vi "loadGraph.vi"(1 "filePath":path, 2 "graphics":refnum<class "Graphics.lvclass">, 3 "grid":refnum<class "Grid.lvclass">, 5 "error in (no error)":errorcluster) -> (14 "reference out":refnum<class "Graph.lvclass">, 15 "succeeded":bool, 16 "String":string, 17 "NodesBounds":T1 {"height" format="%.2f"; "width" format="%.2f"; "y" format="%.2f"; "x" format="%.2f"}, 19 "error out":errorcluster)   [LabVIEW 2020, in "Graph.lvclass"]
doc: "Save to File"
uses:
  <resource>/Framework/Providers/Open_GDS/UML/Graph_class/Graph.lvclass
  <resource>/Framework/Providers/Open_GDS/UML/General/Rectangle/Rectangle Rectangle2D.ctl
  <resource>/Framework/Providers/Open_GDS/UML/Grid_class/Grid.lvclass
  <resource>/Framework/Providers/Open_GDS/UML/Graphics_class/Graphics.lvclass
  <resource>/Framework/Providers/Open_GDS/UML/AbstractNode_class/AbstractNode.lvclass
  <resource>/Framework/Providers/Open_GDS/UML/AbstractEdge_class/AbstractEdge.lvclass
  <resource>/Framework/Providers/Open_GDS/UML/Graph_class/FileContent.ctl
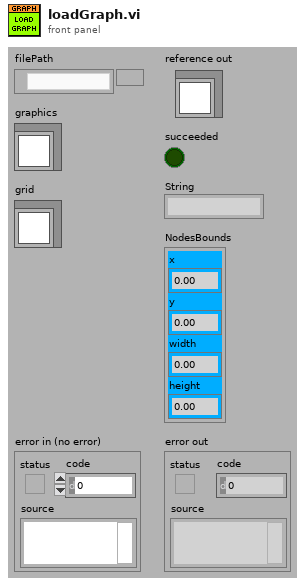
[diagram p1: front panel]
types:
  T1 = typedef "Rectangle Rectangle2D.ctl" = cluster{"x":dbl, "y":dbl, "width":dbl, "height":dbl}
  T2 = cluster{"graph":refnum<class "Graph.lvclass">, "succeeded":bool, "nodeInfo":cluster{"NodeType":string[], "ParentIndex":i32[], "ChildernIndexies":cluster{i32[]}[], "FlattenData":string[]}, "edgeInfo":cluster{"EdgeType":string[], "StartNodeIndex":i32[], "EndNodeIndex":i32[], "FlattenData":string[]}, "nodes":refnum<class "AbstractNode.lvclass">[], "edges":refnum<class "AbstractEdge.lvclass">[], "DiagramData":string, "bounds":T1, "diagramType":string}
  T3 = typedef "Graph.lvclass/FileContent.ctl" = cluster{"Version":string, "DiagramType":string, "DiagramData":string, "Nodes":cluster{"NodeType":string[], "ParentIndex":i32[], "ChildernIndexies":cluster{i32[]}[], "FlattenData":string[]}, "Edges":cluster{"EdgeType":string[], "StartNodeIndex":i32[], "EndNodeIndex":i32[], "FlattenData":string[]}}
  T4 = enum16{"read/write", "read-only", "write-only", "write-only (truncate)"}
  T5 = enum16{"None", "Class", "Sequency", "State", "UseCase"}
  T6 = cluster{"NodeType":string[], "ParentIndex":i32[], "ChildernIndexies":cluster{i32[]}[], "FlattenData":string[]}
  T7 = cluster{"EdgeType":string[], "StartNodeIndex":i32[], "EndNodeIndex":i32[], "FlattenData":string[]}
  T8 = cluster{"TYPEDEF-FileSaveVersion":enum16{"A"}, "diagramType":enum16{"None", "Class", "Sequency", "State", "UseCase"}, string, "nodeInfo":cluster{"NodeType":string[], "ParentIndex":i32[], "ChildernIndexies":cluster{i32[]}[], "FlattenData":string[]}, "edgeInfo":cluster{"EdgeType":string[], "StartNodeIndex":i32[], "EndNodeIndex":i32[], "FlattenData":string[]}}
  T9 = cluster{"diagramType":enum16{"None", "Class", "Sequency", "State", "UseCase"}, "nodeInfo":cluster{"NodeType":string[], "ParentIndex":i32[], "ChildernIndexies":cluster{i32[]}[], "FlattenData":string[]}, "edgeInfo":cluster{"EdgeType":string[], "StartNodeIndex":i32[], "EndNodeIndex":i32[], "FlattenData":string[]}}
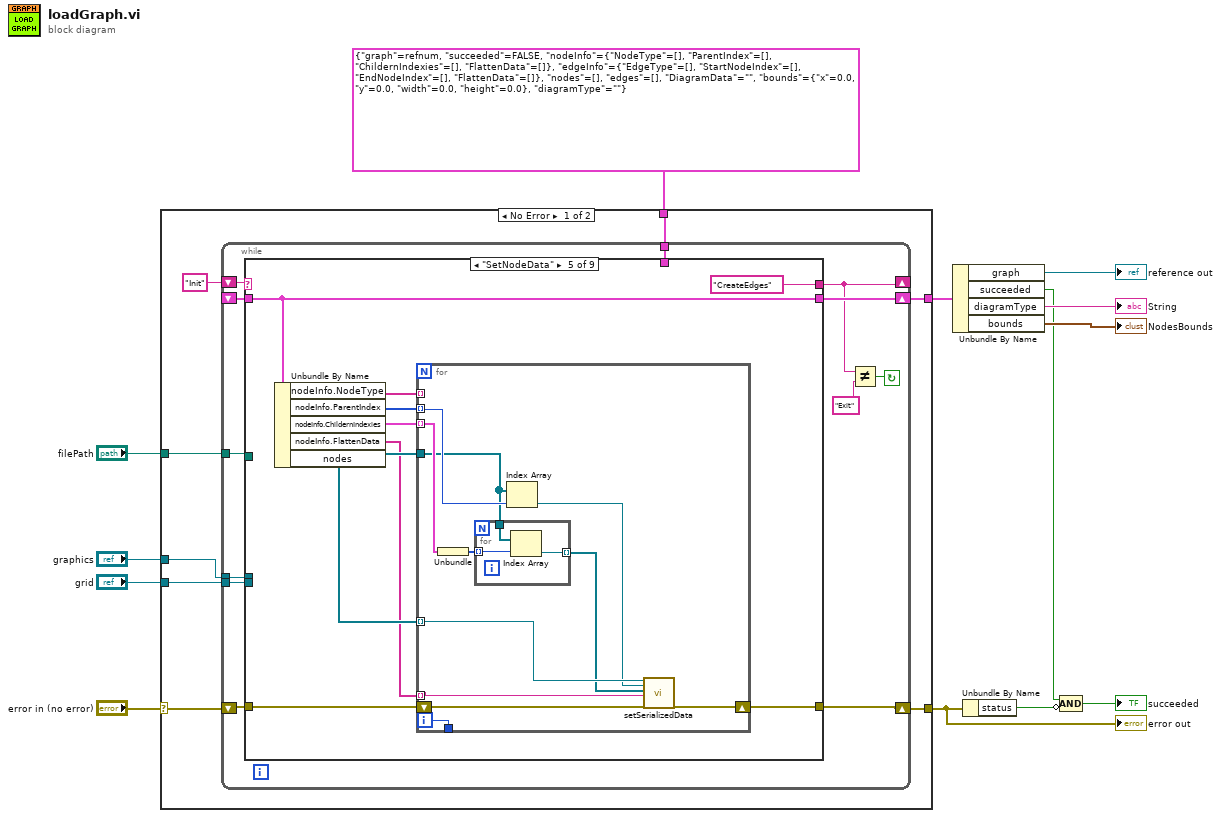
[diagram p0: block diagram]
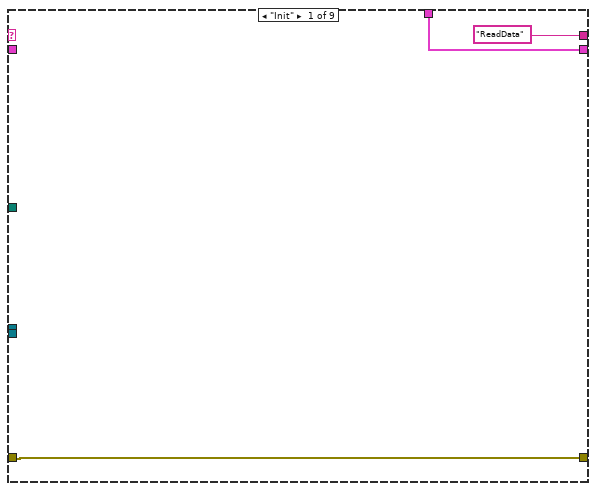
[diagram p2: hidden frame]
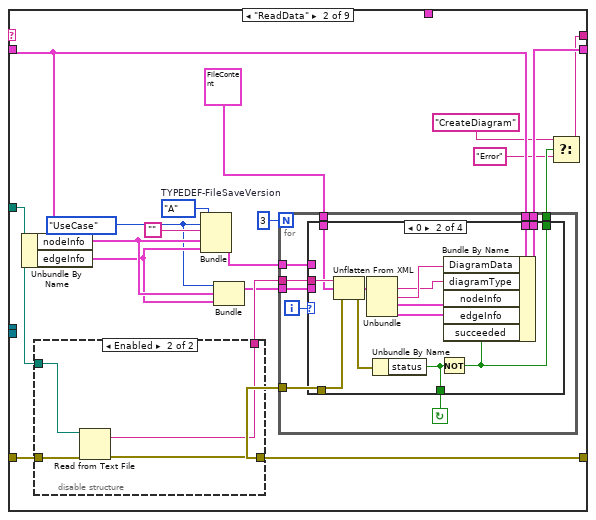
[diagram p3: hidden frame]
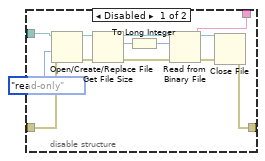
[diagram p4: hidden frame]
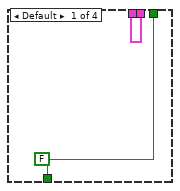
[diagram p5: hidden frame]
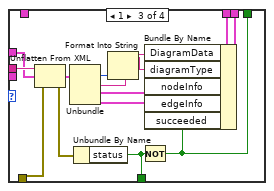
[diagram p6: hidden frame]
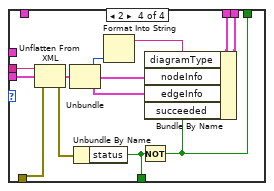
[diagram p7: hidden frame]
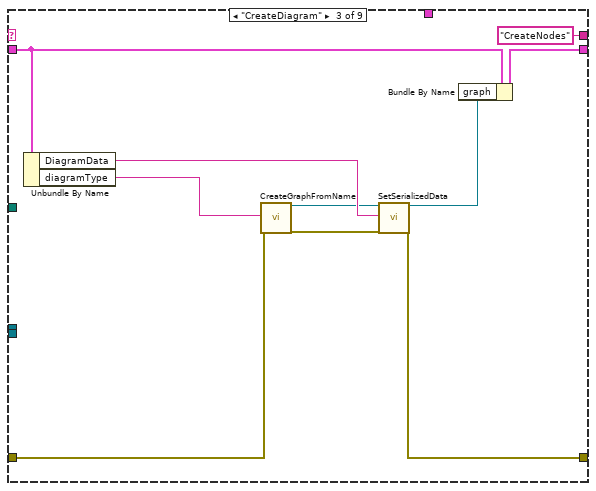
[diagram p8: hidden frame]
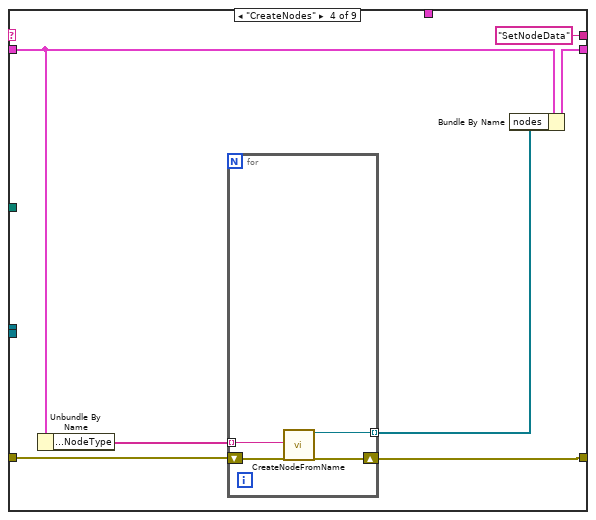
[diagram p9: hidden frame]
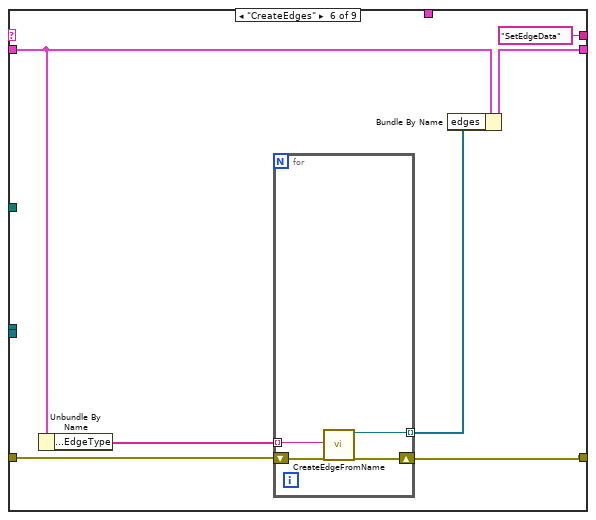
[diagram p10: hidden frame]
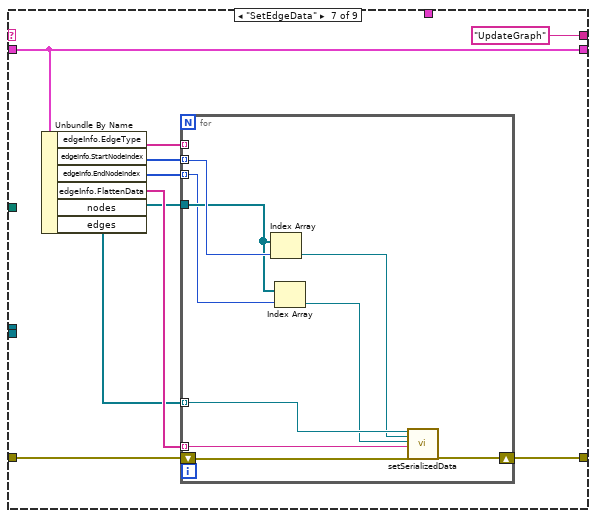
[diagram p11: hidden frame]
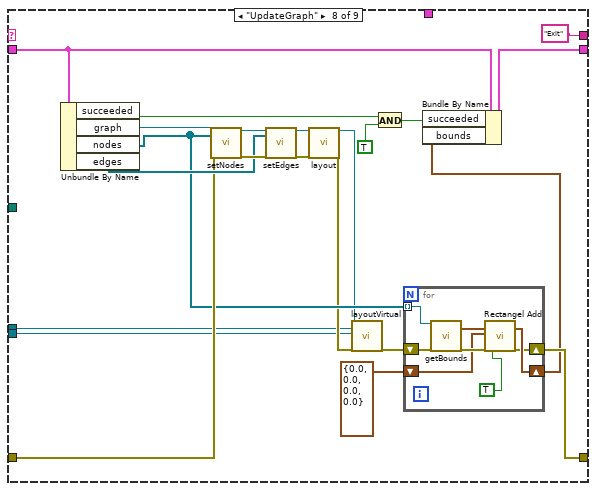
[diagram p12: hidden frame]
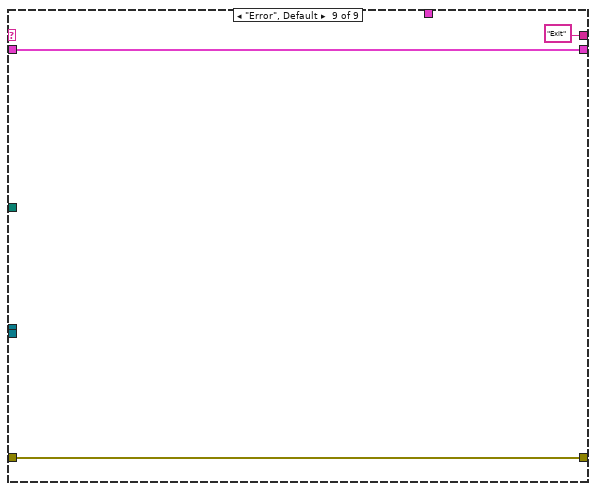
[diagram p13: hidden frame]
diagram:
  n1 = case shown="No Error" "error in (no error)" {
    selector: "error in (no error)" -> [w18 w232]
    tunnel: [w17 w232] -> w5
    tunnel: "filePath" -> [w21 _]
    tunnel: [w19 _] -> w11
    tunnel: "graphics" -> [w16 _]
    tunnel: "grid" -> [w15 _]
    tunnel: T2 {"graph"=refnum, "succeeded"=FALSE, "nodeInfo"={"NodeType"=[], "ParentIndex"=[], "ChildernIndexies"=[], "FlattenData"=[]}, "edgeInfo"={"EdgeType"=[], "StartNodeIndex"=[], "EndNodeIndex"=[], "FlattenData"=[]}, "nodes"=[], "edges"=[], "DiagramData"="", "bounds"={"x"=0.0, "y"=0.0, "width"=0.0, "height"=0.0}, "diagramType"=""} ("localData") -> [w14 _]
    frame No Error {
      n2 = while {
        tunnel: w21 -> [w33]
        shift-right: [w28] -> _
        shift-left: "Init" -> [w32]
        shift-right: [w31] -> w19
        shift-left: _ -> [w27]
        shift-right: [w25] -> w17
        shift-left: w18 -> [w26]
        tunnel: w16 -> [w24]
        tunnel: w15 -> [w23]
        tunnel: w14 -> [w22]
        stop <- w29 continue-if-true
        n3 = case shown="\"SetNodeData\"" w32 {
          tunnel: w26 -> [w36 w48 w128 w139 w147 w173 w183 w214 w231]
          tunnel: w33 -> [_ w47 _ _ _ _ _ _ _]
          tunnel: [w36 w54 w130 w135 w146 w170 w182 w206 w231] -> w25
          tunnel: [w34 w52 w132 w137 w154 w172 w189 w212 w229] -> w31
          tunnel: ["ReadData" w49 "CreateNodes" "SetNodeData" "CreateEdges" ("y") "SetEdgeData" "UpdateGraph" ("y") "Exit" ("y") "Exit" ("y")] -> w28
          tunnel: w27 -> [_ w51 w133 w136 w154 w171 w189 w211 w229]
          tunnel: w24 -> [_ _ _ _ _ _ _ w200 _]
          tunnel: w23 -> [_ _ _ _ _ _ _ w199 _]
          tunnel: w22 -> [w34 _ _ _ _ _ _ _ _]
          frame "Init" {
          }
          frame "ReadData" {
            w43 = enum16{"A"}."A"  # TYPEDEF-FileSaveVersion
            w38 = T5."UseCase" ("diagramType")
            n4 = Unbundle By Name(w51) -> ("nodeInfo"=w41:T6, "edgeInfo"=w40:T7)
            n5 = disable-structure shown="Enabled" {
              disable-tunnel: [w60 w69] -> w55
              disable-tunnel: [w59 w70] -> w54
              disable-tunnel: w48 -> [w58 w72]
              disable-tunnel: w47 -> [w57 w71]
              frame Disabled {
                n6 = Open/Create/Replace File(file path (use dialog)=w57, error in=w58, access (0:read/write)=T4."read-only" ("open mode (0)")) -> (refnum out=w63:refnum<file>, error out=w64:errorcluster)  [unwired: 3 in, 1 out]
                n7 = Get File Size(file=w63, error in=w64) -> (refnum out=w65:refnum<file>, size (in bytes)=w56:i64, 0:w66:errorcluster)
                n8 = To Long Integer(number=w56) -> (32bit integer=w62:i32)
                n9 = Read from Binary File(8:w66, 10:w62, 11:w65) -> (0:w68:errorcluster, 2:w60:string, 3:w67:refnum<file>)  [unwired: 4 out]
                n10 = Close File(refnum=w67, error in=w68) -> (error out=w59:errorcluster)  [unwired: 1 out]
              }
              frame Enabled {
                n11 = Read from Text File(file (use dialog)=w71, error in=w72) -> (text=w69:string, error out=w70:errorcluster)  [unwired: 2 in, 2 out]
              }
            }
            n12 = Bundle("TYPEDEF-FileSaveVersion"=w43, "diagramType"=w38, "", "nodeInfo"=w41, "edgeInfo"=w40) -> (w42:T8)  [unwired: 1 out]
            n13 = Bundle("diagramType"=w38, "nodeInfo"=w41, "edgeInfo"=w40) -> (w53:T9)  [unwired: 1 out]
            n14 = for {
              N: 3 -> [_]
              tunnel: w55 -> [w82]
              tunnel: w54 -> [w81]
              tunnel: w53 -> [w80]
              tunnel: [w79] -> w52
              tunnel: w51 -> [w78]
              tunnel: [w77] -> w50
              tunnel: w42 -> [w75]
              tunnel: T3 {"Version"="", "DiagramType"="", "DiagramData"="", "Nodes"={"NodeType"=[], "ParentIndex"=[], "ChildernIndexies"=[], "FlattenData"=[]}, "Edges"={"EdgeType"=[], "StartNodeIndex"=[], "EndNodeIndex"=[], "FlattenData"=[]}} ("cluster") -> [w73]
              i -> [w76]
              stop <- w74 continue-if-true
              n15 = case shown="0" w76 {
                tunnel: w82 -> [_ w97 w111 w124]
                tunnel: w81 -> [_ w96 w110 w123]
                tunnel: w80 -> [_ _ _ w121]
                tunnel: [w84 w94 w108 w118] -> w79
                tunnel: w78 -> [w84 w93 w107 w117]
                tunnel: [w83 w90 w104 w114] -> w77
                tunnel: [w83 w91 w105 w115] -> w74
                tunnel: w75 -> [_ _ w103 _]
                tunnel: w73 -> [_ w86 _ _]
                frame Default {
                  w83 = FALSE ("status")
                }
                frame 0 {
                  n16 = Unflatten From XML(xml string=w97, type=w86, error in (no error)=w96) -> (value=w95:T3, error out=w92:errorcluster)
                  n17 = Unbundle(w95) -> ("DiagramType"=w85:string, "DiagramData"=w87:string, "Nodes"=w89:T6, "Edges"=w88:T7)  [unwired: 1 out]
                  n18 = Unbundle By Name(w92) -> ("status"=w91:bool)
                  n19 = Not(x=w91) -> (.not. x?=w90:bool)
                  n20 = Bundle By Name(cluster=w93, "DiagramData"=w87, "diagramType"=w85, "nodeInfo"=w89, "edgeInfo"=w88, "succeeded"=w90) -> (w94:T2)
                }
                frame 1 {
                  n21 = Unflatten From XML(xml string=w111, type=w103, error in (no error)=w110) -> (value=w109:T8, error out=w106:errorcluster)
                  n22 = Unbundle(w109) -> ("diagramType"=w99:T5, w100:string, "nodeInfo"=w102:T6, "edgeInfo"=w101:T7)  [unwired: 1 out]
                  n23 = Unbundle By Name(w106) -> ("status"=w105:bool)
                  n24 = Format Into String(w99) -> (resulting string=w98:string)  [unwired: 3 in, 1 out]
                  n25 = Not(x=w105) -> (.not. x?=w104:bool)
                  n26 = Bundle By Name(cluster=w107, "DiagramData"=w100, "diagramType"=w98, "nodeInfo"=w102, "edgeInfo"=w101, "succeeded"=w104) -> (w108:T2)
                }
                frame 2 {
                  n27 = Unflatten From XML(xml string=w124, type=w121, error in (no error)=w123) -> (value=w122:T9, error out=w116:errorcluster)
                  n28 = Unbundle(w122) -> ("diagramType"=w113:T5, "nodeInfo"=w120:T6, "edgeInfo"=w119:T7)
                  n29 = Unbundle By Name(w116) -> ("status"=w115:bool)
                  n30 = Format Into String(w113) -> (resulting string=w112:string)  [unwired: 3 in, 1 out]
                  n31 = Not(x=w115) -> (.not. x?=w114:bool)
                  n32 = Bundle By Name(cluster=w117, "diagramType"=w112, "nodeInfo"=w120, "edgeInfo"=w119, "succeeded"=w114) -> (w118:T2)
                }
              }
            }
            n33 = Select(t="CreateDiagram" ("y"), s=w50, f="Error" ("y")) -> (s? t:f=w49:string)
          }
          frame "CreateDiagram" {
            n34 = Unbundle By Name(w133) -> ("DiagramData"=w131:string, "diagramType"=w125:string)
            n35 = call <resource>:"CreateGraphFromName.vi"("GraphTypeToCreate"=w125, "error in (no error)"=w128) -> ("GraphCreated"=w126:refnum<class "Graph.lvclass">, "error out"=w127:errorcluster)  [unwired: 16 in]
            n36 = call-dynamic "SetSerializedData.vi"("reference in"=w126, "SerializedData(XML)"=w131, "error in (no error)"=w127) -> ("reference out"=w129:refnum<class "Graph.lvclass">, "error out"=w130:errorcluster)  [unwired: 15 in]
            n37 = Bundle By Name(cluster=w133, "graph"=w129) -> (w132:T2)
          }
          frame "CreateNodes" {
            n38 = Unbundle By Name(w136) -> ("nodeInfo.NodeType"=w140:string[])
            n39 = for {
              tunnel: w140 -> [w145] mode=indexing
              shift-right: [w143] -> w135
              shift-left: w139 -> [w144]
              tunnel: [w142] -> w138 mode=indexing
              n40 = call <resource>:"CreateNodeFromName.vi"("NodeTypeToCreate"=w145, "error in (no error)"=w144) -> ("NodeCreated"=w142:refnum<class "AbstractNode.lvclass">, "error out"=w143:errorcluster)  [unwired: 16 in]
            }
            n41 = Bundle By Name(cluster=w136, "nodes"=w138) -> (w137:T2)
          }
          frame "SetNodeData" {
            n42 = Unbundle By Name(w154) -> ("nodeInfo.NodeType"=w152:string[], "nodeInfo.ParentIndex"=w151:i32[], "nodeInfo.ChildernIndexies"=w150:cluster{i32[]}[], "nodeInfo.FlattenData"=w148:string[], "nodes"=w149:refnum<class "AbstractNode.lvclass">[])
            n43 = for {
              tunnel: w152 -> [_] mode=indexing
              tunnel: w151 -> [w165] mode=indexing
              tunnel: w150 -> [w164] mode=indexing
              tunnel: w149 -> [w163]
              tunnel: w149 -> [w161] mode=indexing
              tunnel: w148 -> [w157] mode=indexing
              shift-right: [w158] -> w146
              shift-left: w147 -> [w156]
              tunnel: [w155] -> _
              i -> [w155]
              n44 = Unbundle(w164) -> (w162:i32[])
              n45 = for {
                tunnel: w163 -> [w168]
                tunnel: w162 -> [w167] mode=indexing
                tunnel: [w166] -> w159 mode=indexing
                n46 = Index Array(array=w168, index=w167) -> (element=w166:refnum<class "AbstractNode.lvclass">)
              }
              n47 = Index Array(array=w163, index=w165) -> (element=w160:refnum<class "AbstractNode.lvclass">)
              n48 = call-dynamic "setSerializedData.vi"("reference"=w161, "parent"=w160, "children"=w159, "xmlOut"=w157, "error in (no error)"=w156) -> ("error out"=w158:errorcluster)  [unwired: 13 in, 1 out]
            }
          }
          frame "CreateEdges" {
            n49 = Unbundle By Name(w171) -> ("edgeInfo.EdgeType"=w174:string[])
            n50 = for {
              tunnel: w174 -> [w176] mode=indexing
              shift-right: [w179] -> w170
              shift-left: w173 -> [w177]
              tunnel: [w178] -> w169 mode=indexing
              n51 = call <resource>:"CreateEdgeFromName.vi"("NodeTypeToCreate"=w176, "error in (no error)"=w177) -> ("AbstractCreated"=w178:refnum<class "AbstractEdge.lvclass">, "error out"=w179:errorcluster)  [unwired: 16 in]
            }
            n52 = Bundle By Name(cluster=w171, "edges"=w169) -> (w172:T2)
          }
          frame "SetEdgeData" {
            n53 = Unbundle By Name(w189) -> ("edgeInfo.EdgeType"=w187:string[], "edgeInfo.StartNodeIndex"=w186:i32[], "edgeInfo.EndNodeIndex"=w185:i32[], "edgeInfo.FlattenData"=w184:string[], "nodes"=w181:refnum<class "AbstractNode.lvclass">[], "edges"=w180:refnum<class "AbstractEdge.lvclass">[])
            n54 = for {
              tunnel: w187 -> [_] mode=indexing
              tunnel: w186 -> [w198] mode=indexing
              tunnel: w185 -> [w192] mode=indexing
              tunnel: w181 -> [w197]
              tunnel: w180 -> [w196] mode=indexing
              tunnel: w184 -> [w191] mode=indexing
              shift-right: [w193] -> w182
              shift-left: w183 -> [w190]
              n55 = Index Array(array=w197, index=w198) -> (element=w195:refnum<class "AbstractNode.lvclass">)
              n56 = Index Array(array=w197, index=w192) -> (element=w194:refnum<class "AbstractNode.lvclass">)
              n57 = call-dynamic "setSerializedData.vi"("reference"=w196, "startNode"=w195, "endNode"=w194, "xmlOut"=w191, "error in (no error)"=w190) -> ("error out"=w193:errorcluster)  [unwired: 13 in, 1 out]
            }
          }
          frame "UpdateGraph" {
            n58 = Unbundle By Name(w211) -> ("succeeded"=w210:bool, "graph"=w220:refnum<class "Graph.lvclass">, "nodes"=w205:refnum<class "AbstractNode.lvclass">[], "edges"=w217:refnum<class "AbstractEdge.lvclass">[])
            n59 = call-dynamic "setNodes.vi"("reference"=w220, "nodes"=w205, "error in (no error)"=w214) -> ("reference out"=w219:refnum<class "Graph.lvclass">, "error out"=w218:errorcluster)  [unwired: 15 in]
            n60 = call-dynamic "setEdges.vi"("reference"=w219, "edges"=w217, "error in (no error)"=w218) -> ("reference out"=w216:refnum<class "Graph.lvclass">, "error out"=w215:errorcluster)  [unwired: 15 in]
            n61 = call-dynamic "layout.vi"("reference"=w216, "error in (no error)"=w215) -> ("reference out"=w202:refnum<class "Graph.lvclass">, "error out"=w201:errorcluster)  [unwired: 16 in]
            n62 = call <resource>:"layoutVirtual.vi"("reference"=w202, "graphics"=w200, "grid"=w199, "error in (no error)"=w201) -> ("error out"=w203:errorcluster)  [unwired: 15 out]
            n63 = And(x=w210, y=TRUE) -> (x .and. y?=w209:bool)
            n64 = for {
              shift-right: [w223] -> w206
              shift-left: w203 -> [w222]
              shift-right: [w224] -> w204
              shift-left: T1 {"x"=0.0, "y"=0.0, "width"=0.0, "height"=0.0} ("boundsAdded") -> [w225]
              tunnel: w205 -> [w221] mode=indexing
              n65 = call-dynamic "getBounds.vi"("reference"=w221, "error in (no error)"=w222) -> ("bounds"=w228:T1, "error out"=w227:errorcluster)  [unwired: 15 in, 1 out]
              n66 = call <resource>:"Rectangel Add.vi"("bounds1"=w228, "bounds2"=w225, "error in (no error)"=w227, "useAbsoluteCordinates(False)"=TRUE) -> ("boundsAdded"=w224:T1, "error out"=w223:errorcluster)  [unwired: 1 in, 13 out]
            }
            n67 = Bundle By Name(cluster=w211, "succeeded"=w209, "bounds"=w204) -> (w212:T2)
          }
          frame "Error", Default {
          }
        }
        n68 = Not Equal?(x=w28, y="Exit") -> (x != y?=w29:bool)
      }
    }
    frame Error {
    }
  }
  "error out" <- w5
  n69 = Unbundle By Name(w11) -> ("graph"=→"reference out":refnum<class "Graph.lvclass">, "succeeded"=w3:bool, "diagramType"=→"String":string, "bounds"=→"NodesBounds":T1)
  n70 = Unbundle By Name(w5) -> ("status"=w4:bool)
  n71 = Compound Arithmetic op=AND(w3, invert w4) -> (→"succeeded":bool)
